vi "SNR_Symbols1.vi"(10 "Ideal Symbols":cdb[](array[numeric]), 11 "Received symbols":cdb[](array[numeric])) -> (3 "SNR dB":dbl)   [LabVIEW 2022 SP3]
uses:
  <vilib>/Analysis/baseanly.llb/Mean (DBL).vi
  <vilib>/Analysis/NI_AALBase.lvlib
panel:
  out "SNR valid?":bool
  out "size(s)":i32
  out "size(s) 2":i32
  out "P_error":dbl
  out "P_ideal":dbl
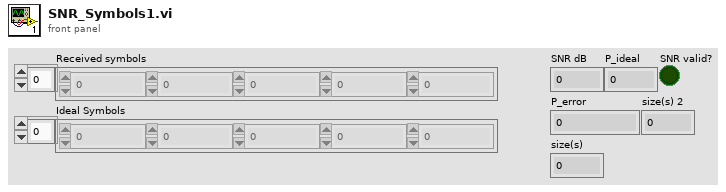
[diagram p1: front panel]
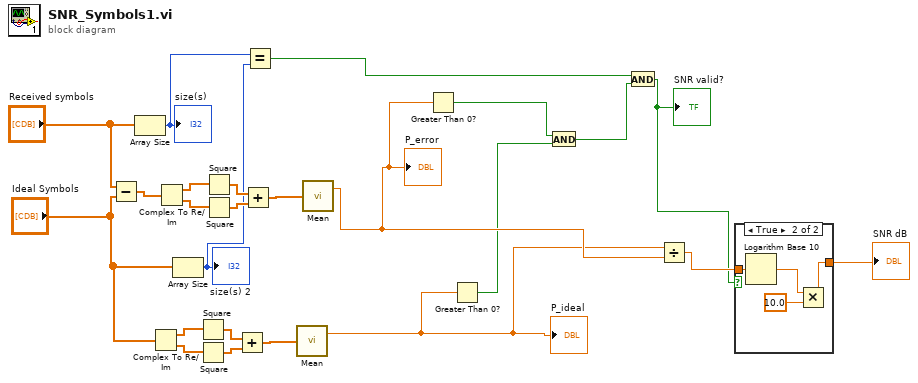
[diagram p0: block diagram]
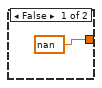
[diagram p2: hidden frame]
diagram:
  n1 = Subtract(x="Received symbols", y="Ideal Symbols") -> (x-y=w24:cdb[])
  n2 = Array Size(array="Received symbols") -> (size(s)=w5:i32)
  "size(s)" <- w5
  n3 = Complex To Re/Im(x + iy="Ideal Symbols") -> (x=w18:dbl[], y=w17:dbl[])
  n4 = Complex To Re/Im(x + iy=w24) -> (x=w23:dbl[], y=w22:dbl[])
  n5 = Array Size(array="Ideal Symbols") -> (size(s)=w4:i32)
  "size(s) 2" <- w4
  n6 = Square(x=w18) -> (x^2=w16:dbl[])
  n7 = Square(x=w17) -> (x^2=w15:dbl[])
  n8 = Square(x=w23) -> (x^2=w21:dbl[])
  n9 = Square(x=w22) -> (x^2=w20:dbl[])
  n10 = Add(x=w16, y=w15) -> (x+y=w14:dbl[])
  n11 = Add(x=w21, y=w20) -> (x+y=w19:dbl[])
  n12 = Equal?(x=w5, y=w4) -> (x = y?=w3:bool)
  n13 = call-poly <vilib>:"Mean.vi"("X"=w14) -> ("mean"=w8:dbl)  [unwired: 1 out]
  "P_ideal" <- w8
  n14 = call-poly <vilib>:"Mean.vi"("X"=w19) -> ("mean"=w9:dbl)  [unwired: 1 out]
  "P_error" <- w9
  n15 = Greater Than 0?(x=w9) -> (x > 0?=w7:bool)
  n16 = Greater Than 0?(x=w8) -> (x > 0?=w6:bool)
  n17 = And(x=w7, y=w6) -> (x .and. y?=w2:bool)
  n18 = And(x=w3, y=w2) -> (x .and. y?=w1:bool)
  "SNR valid?" <- w1
  n19 = Divide(x=w8, y=w9) -> (x/y=w12:dbl)
  n20 = case shown="True" w1 {
    tunnel: [nan w26] -> w13
    tunnel: w12 -> [_ w27]
    frame False {
    }
    frame True {
      n21 = Logarithm Base 10(1:w27) -> (0:w29:dbl)
      n22 = Multiply(x=w29, y=10.0) -> (x*y=w26:dbl)
    }
  }
  "SNR dB" <- w13
